vi "_Start VI Helpeks.vi"   [LabVIEW 2014]
doc: "::: VI Helpeks :::\nCopyright (c) 2000-2026 Konstantin Shifershteyn. All rights reserved."
types:
  T1 = enum32{"Invalid", "Standard", "Closed", "Hidden", "Minimized", "Maximized"}
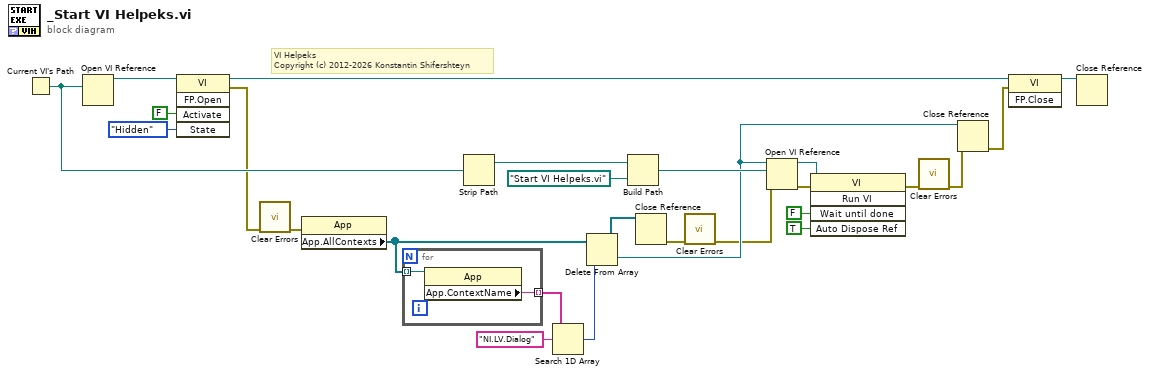
[diagram p0: block diagram]
diagram:
  # "VI Helpeks\nCopyright (c) 2012-2026 Konstantin Shifershteyn"
  n1 = Current VI's Path() -> (path=w24:path)
  n2 = Open VI Reference(vi path=w24) -> (vi reference=w8:refnum<vi>)  [unwired: 5 in, 1 out]
  n3 = invoke class="VI" method="FP.Open"(reference=w8, "Activate"=FALSE ("Activate?"), "State"=T1."Hidden") -> (reference out=w3:refnum<vi>, error out=w6:errorcluster)  [unwired: 2 in, 3 out]
  n4 = call <vilib>:"Clear Errors.vi"("error in (no error)"=w6) -> ("error out"=w7:errorcluster)  [unwired: 5 in, 1 out]
  n5 = property class="App"(error in=w7) -> ("App.AllContexts"=w21:refnum<vi>[])  [unwired: 1 in, 2 out]
  n6 = for {
    tunnel: w21 -> [w28] mode=indexing
    tunnel: [w27] -> w19 mode=indexing
    n7 = property class="App"(reference=w28) -> ("App.ContextName"=w27:string)  [unwired: 1 in, 2 out]
  }
  n8 = Strip Path(path=w24) -> (stripped path=w25:path)  [unwired: 1 out]
  n9 = Search 1D Array(1D array=w19, element="NI.LV.Dialog") -> (index of element=w22:i32)  [unwired: 1 in]
  n10 = Delete From Array(array=w21, index=w22) -> (deleted portion=w11:refnum<vi>, array with subset deleted=w23:refnum<vi>[])  [unwired: 1 in]
  n11 = Build Path(base path=w25, name or relative path=path "Start VI Helpeks.vi") -> (appended path=w18:path)
  n12 = Close Reference(reference=w23) -> (error out=w10:errorcluster)  [unwired: 1 in]
  n13 = call <vilib>:"Clear Errors.vi"("error in (no error)"=w10) -> ("error out"=w9:errorcluster)  [unwired: 5 in, 1 out]
  n14 = Open VI Reference(application reference (local)=w11, vi path=w18, error in (no error)=w9) -> (vi reference=w17:refnum<vi>, error out=w16:errorcluster)  [unwired: 3 in]
  n15 = invoke class="VI" method="Run VI"(reference=w17, error in=w16, "Wait until done"=FALSE ("Wait Until Done"), "Auto Dispose Ref"=TRUE ("Auto Dispose Reference")) -> (error out=w14:errorcluster)  [unwired: 1 in, 4 out]
  n16 = call <vilib>:"Clear Errors.vi"("error in (no error)"=w14) -> ("error out"=w12:errorcluster)  [unwired: 5 in, 1 out]
  n17 = Close Reference(reference=w11, error in (no error)=w12) -> (error out=w1:errorcluster)
  n18 = invoke class="VI" method="FP.Close"(reference=w3, error in=w1) -> (reference out=w2:refnum<vi>)  [unwired: 1 in, 2 out]
  n19 = Close Reference(reference=w2) -> ()  [unwired: 1 in, 1 out]
